vi "Select Preview Channel.vi"(6 "Host Resources in":T10, 9 "Channel to Preview":string, 10 "Previous Selected Channel":i32, 11 "Hardware Configuration":T1) -> (0 "Selected Channel":T2, 1 "Selected Channel Changed?":bool, 2 "Selected Channel Index":i32, 3 "Hardware Configuration for Preview Channel":T1)   [LabVIEW 2021, in "Settings.lvlib"]
doc: "Get the index of the channel that has the name 'Channel to Preview' from the 'Hardware Configuration' array. Isolate that matched channel as the only channel in 'Hardware Configuration for Preview Channel' and select the supporting API. If the index is different from the previous one, return True for 'Selected Channel Changed?'"
uses:
  Settings.lvlib
  Acquisition/Channel Settings.ctl
  Acquisition/IO Device.ctl
  Acquisition/Sensor Type.ctl
  Acquisition/Host Resources.ctl
  Acquisition/Host Software Package.ctl
  Acquisition/Host IO Resource.ctl
  Acquisition/Hardware Configuration.ctl
  Interval Timer/Repeat Interval.ctl
  Interval Timer/Interval Length.ctl
  Interval Timer/Interval Token.ctl
  Acquisition/IO Context.ctl
  Acquisition/IO API.ctl
  Acquisition/Acquisition.lvlib
  Interval Timer/Interval Timer.lvlib
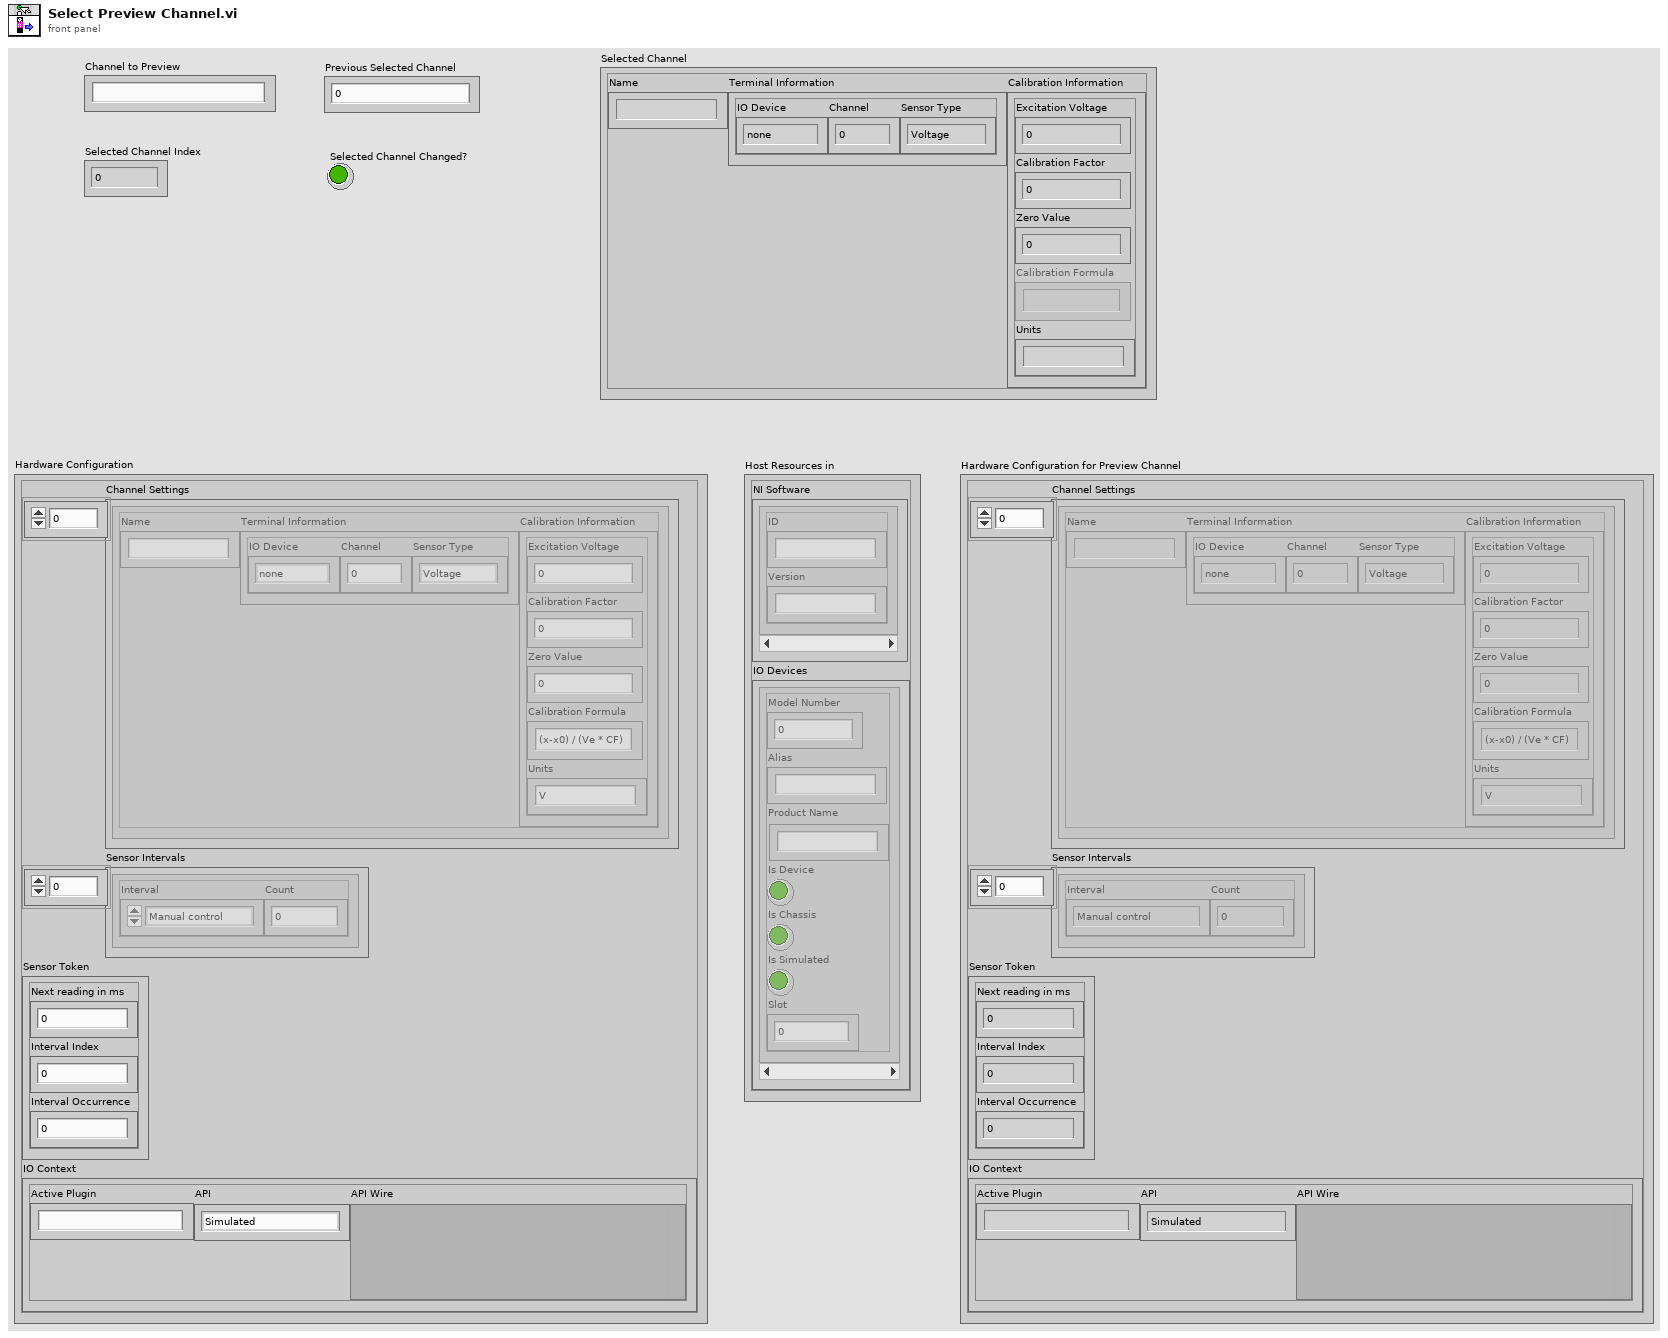
[diagram p1: front panel]
types:
  T1 = typedef "Acquisition.lvlib/Hardware Configuration.ctl" = cluster{"Channel Settings":T2[], "Sensor Intervals":T5[], "Sensor Token":T7, "IO Context":T8}
  T2 = typedef "Acquisition.lvlib/Channel Settings.ctl" = cluster{"Name":string, "Terminal Information":cluster{"IO Device":T3, "Channel":i32, "Sensor Type":T4}, "Calibration Information":cluster{"Excitation Voltage":dbl, "Calibration Factor":dbl, "Zero Value":dbl, "Calibration Formula":string, "Units":string}}
  T3 = typedef "Acquisition.lvlib/IO Device.ctl" = enum16{"none", "9219", "9401"}
  T4 = typedef "Acquisition.lvlib/Sensor Type.ctl" = enum16{"Voltage", "Load", "Pressure", "Encoder"}
  T5 = typedef "Interval Timer.lvlib/Repeat Interval.ctl" = cluster{"Interval":T6, "Count":i32}
  T6 = typedef "Interval Timer.lvlib/Interval Length.ctl" = enum16{"Manual control", "1 second", "10 seconds", "30 seconds", "60 seconds", "600 seconds", "1200 seconds", "3600 seconds"}
  T7 = typedef "Interval Timer.lvlib/Interval Token.ctl" = cluster{"Next reading in ms":u32, "Interval Index":i32, "Interval Occurrence":i32}
  T8 = typedef "Acquisition.lvlib/IO Context.ctl" = cluster{"Active Plugin":string, "API":T9, "API Wire":variant}
  T9 = typedef "Acquisition.lvlib/IO API.ctl" = enum16{"Simulated", "DAQmx"}
  T10 = typedef "Acquisition.lvlib/Host Resources.ctl" = cluster{"NI Software":T11[], "IO Devices":T12[]}
  T11 = typedef "Acquisition.lvlib/Host Software Package.ctl" = cluster{"ID":string, "Version":string}
  T12 = typedef "Acquisition.lvlib/Host IO Resource.ctl" = cluster{"Model Number":u32, "Alias":string, "Product Name":string, "Is Device":bool, "Is Chassis":bool, "Is Simulated":bool, "Slot":i32}
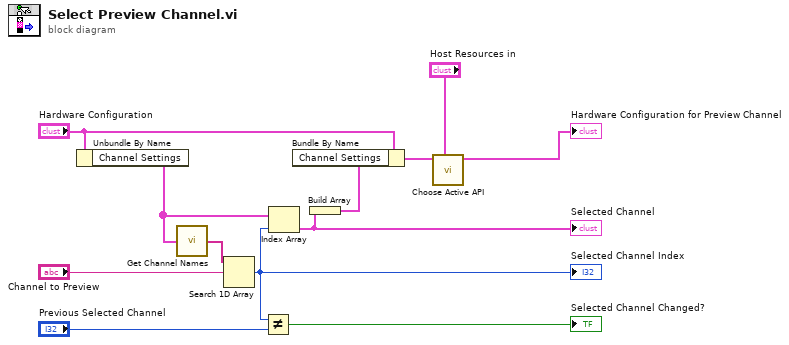
[diagram p0: block diagram]
diagram:
  n1 = Unbundle By Name("Hardware Configuration") -> ("Channel Settings"=w2:T2[])
  n2 = call "Get Channel Names.vi"("Channel Settings"=w2) -> ("Channel Names"=w12:string[])
  n3 = Search 1D Array(1D array=w12, element="Channel to Preview") -> (index of element=w8:i32)  [unwired: 1 in]
  "Selected Channel Index" <- w8
  n4 = Not Equal?(x=w8, y="Previous Selected Channel") -> (x != y?=→"Selected Channel Changed?":bool)
  n5 = Index Array(array=w2, index=w8) -> (element=w1:T2)
  "Selected Channel" <- w1
  n6 = Build Array(w1) -> (w3:T2[])
  n7 = Bundle By Name(cluster="Hardware Configuration", "Channel Settings"=w3) -> (w5:T1)
  n8 = call "Choose Active API.vi"("Host Resources"="Host Resources in", "Hardware Configuration in"=w5) -> ("Hardware Configuration out"=→"Hardware Configuration for Preview Channel":T1)  [unwired: 9 in]
